vi "Two Way Event Recorder Property Lookup.vi"() -> ()   [LabVIEW 2017, in "Two Way Event Recorder Custom Device.lvlib"]
uses:
  Two Way Event Recorder Custom Device.lvlib
panel:
  in  "Timeout (mS)":string="Timeout"
  in  "Visa Ref":string="Visa Ref"
  in  "Flow Control":string="Flow Control"
  in  "Baud Rate":string="Baud Rate"
  in  "Parity":string="Parity"
  in  "Stop Bit":string="Stop Bit"
  in  "Data Bits":string="Data Bits"
  in  "Start Bit":string="Start Bit"
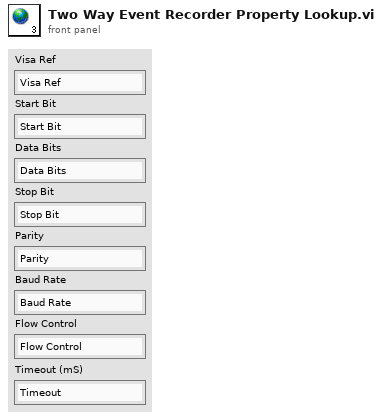
[diagram p1: front panel]
diagram:
